vi "Chrg_Dschrg_PTB.vi"(0 "Data Task in":refnum<k21>, 1 "data task error in":errorcluster, 2 "#DAQ outputs (1-13)":i32, 3 "Battery Type":T1(ring), 4 "PS VISA in 2":refnum<visa-resource-name>, 5 "PS error in 2":errorcluster, 6 "CyclePath 2":path=path "C:/Users/ga11/Desktop/VI/results/3PtestCharge.lvm" caption="Filename", 8 "Charge/discharge 2":enum8{"Charge", "Discharge"}(ring), 9 "Charge/Discharge Voltage Setpoint  2":dbl format="%#.6g", 10 "CC or CCCV 2":enum16{"CC", "CCCV"}(ring), 11 "Current Setpoint 2":dbl format="%#.6g", 13 "Current Cutoff 2":dbl) -> (14 "data task out":refnum<k21>, 15 "data task error out":errorcluster, 18 "PS VISA out":refnum<visa-resource-name>, 19 "PS error out 2":errorcluster)   [LabVIEW 2020]
uses:
  IT-M3400/IT-M3400.lvlib
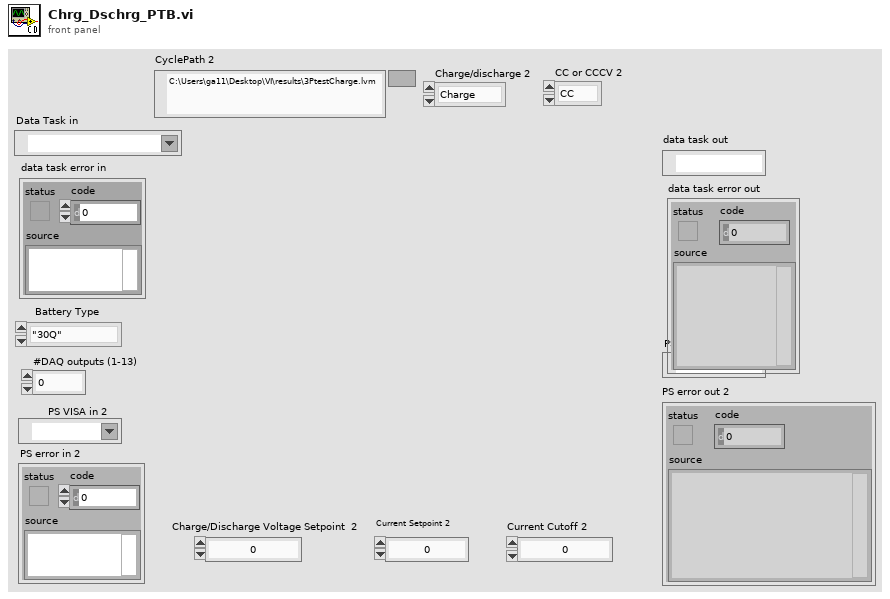
[diagram p1: front panel]
types:
  T1 = enum16{"\"30Q\"", "\"40T\"", "\"2P30Q\"", "\"3P30Q\"", "\"Nissan Leaf\""}
  T2 = cluster{"Baud Rate":u32, "Parity":u16, "Data Bits":u16, "Stop Bits":u16, "Flow Control":u16}
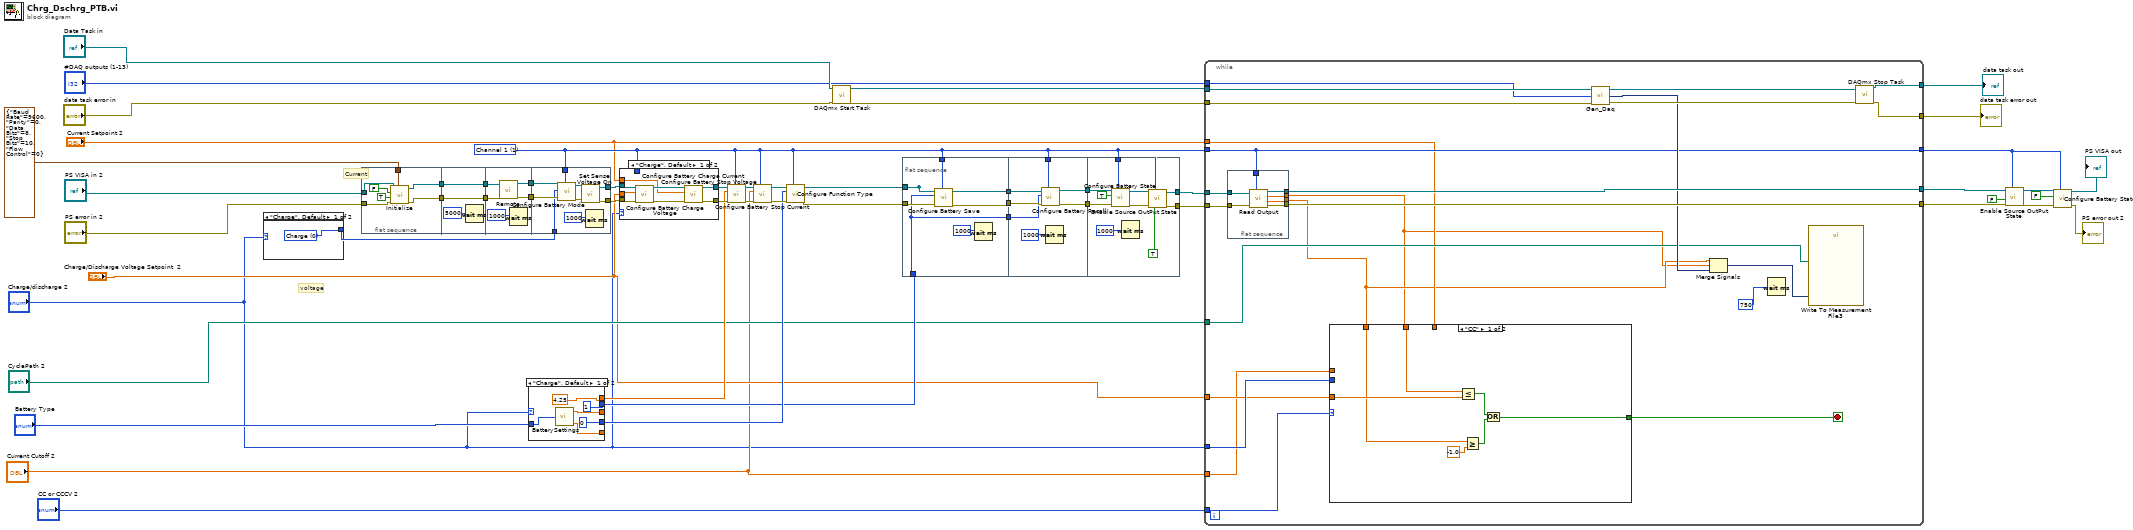
[diagram p0: block diagram]
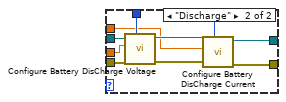
[diagram p2: hidden frame]
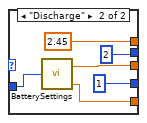
[diagram p3: hidden frame]
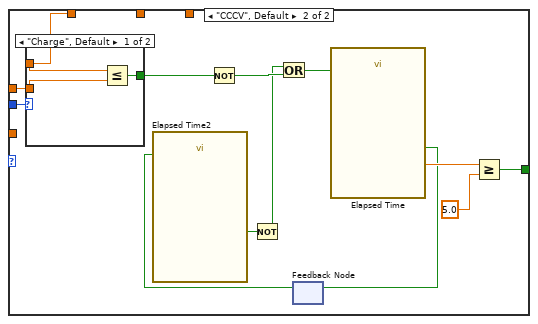
[diagram p4: hidden frame]
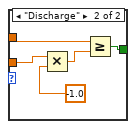
[diagram p5: hidden frame]
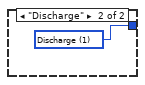
[diagram p6: hidden frame]
diagram:
  w23 = 1 items=["Channel 1"=1, "Channel 2"=2, "Channel 3"=3, "Channel 4"=4, "Channel 5"=5, "Channel 6"=6, "Channel 7"=7, "Channel 8"=8, "Channel 8"=9, "Channel 10"=10, "Channel 11"=11, "Channel 12"=12, "Channel 13"=13, "Channel 14"=14, "Channel 15"=15, "Channel 16"=16] ("Channel")
  # "voltage"
  # "Current"
  n1 = case shown="\"Charge\", Default" "Charge/discharge 2" {
    tunnel: [w55 w56] -> w28
    frame "Charge", Default {
      w55 = u8 0 items=["Charge", "Discharge"] ("Battery Mode")
    }
    frame "Discharge" {
      w56 = u8 1 items=["Charge", "Discharge"] ("Battery Mode")
    }
  }
  n2 = flat-sequence {
    tunnel: [w59] -> w49
    tunnel: [w60] -> w48
    tunnel: T2 {"Baud Rate"=9600, "Parity"=0, "Data Bits"=8, "Stop Bits"=10, "Flow Control"=0} ("Serial Configuration") -> [w63]
    tunnel: "PS error in 2" -> [w62]
    tunnel: "PS VISA in 2" -> [w61]
    tunnel: w49 -> [w66]
    tunnel: [w66] -> w47
    tunnel: w48 -> [w65]
    tunnel: [w65] -> w46
    tunnel: [w71] -> w45
    tunnel: [w70] -> w44
    tunnel: w47 -> [w69]
    tunnel: w46 -> [w68]
    tunnel: w45 -> [w77]
    tunnel: w44 -> [w79]
    tunnel: w23 -> [w80]
    tunnel: w28 -> [w78]
    tunnel: [w72] -> w20
    tunnel: [w73] -> w19
    frame #0 {
      n3 = call "Initialize.vi"("Serial Configuration"=w63, "error in"=w62, "Reset"=TRUE, "ID Query"=FALSE, "VISA resource name"=w61) -> ("error out"=w60:errorcluster, "VISA resource name out"=w59:refnum<visa-resource-name>)  [unwired: 5 in]
    }
    frame #1 {
      n4 = Wait (ms)(milliseconds to wait=5000) -> ()  [unwired: 1 out]
    }
    frame #2 {
      n5 = call "Remote.vi"("error in"=w68, "VISA resource name"=w69) -> ("error out"=w70:errorcluster, "VISA resource name out"=w71:refnum<visa-resource-name>)  [unwired: 8 in]
      n6 = Wait (ms)(milliseconds to wait=1000) -> ()  [unwired: 1 out]
    }
    frame #3 {
      n7 = call "Configure Battery Mode.vi"("Channel"=w80, "error in"=w79, "Battery Mode"=w78, "VISA resource name"=w77) -> ("error out"=w75:errorcluster, "VISA resource name out"=w74:refnum<visa-resource-name>)  [unwired: 6 in]
      n8 = call "Set Sense Voltage On.vi"("error in"=w75, "VISA resource name"=w74) -> ("error out"=w72:errorcluster, "VISA resource name out"=w73:refnum<visa-resource-name>)  [unwired: 8 in]
      n9 = Wait (ms)(milliseconds to wait=1000) -> ()  [unwired: 1 out]
    }
  }
  n10 = case shown="\"Charge\", Default" "Charge/discharge 2" {
    tunnel: [w86 w91] -> _
    tunnel: [u8 0 ("File") u8 1 ("File")] -> w24
    tunnel: [u8 1 ("File") u8 2 ("File")] -> w22
    tunnel: [w83 w89] -> _
    tunnel: [4.25 2.45] -> w21
    tunnel: "Battery Type" -> [w81 w87]
    frame "Charge", Default {
      n11 = call "BatterySettings.vi"("Battery Type"=w81) -> ("RatedCapacity (Ah)"=w83:dbl, "Max Voltage (V)"=w86:dbl)  [unwired: 2 in, 1 out]
    }
    frame "Discharge" {
      n12 = call "BatterySettings.vi"("Battery Type"=w87) -> ("RatedCapacity (Ah)"=w89:dbl, "Min Voltage (V)"=w91:dbl)  [unwired: 2 in, 1 out]
    }
  }
  n13 = case shown="\"Charge\", Default" "Charge/discharge 2" {
    tunnel: w19 -> [w100 w109]
    tunnel: w20 -> [w99 w108]
    tunnel: [w94 w105] -> w35
    tunnel: [w93 w104] -> w34
    tunnel: w23 -> [_ w103]
    tunnel: "Charge/Discharge Voltage Setpoint  2" -> [w96 w102]
    tunnel: "Current Setpoint 2" -> [w95 w101]
    frame "Charge", Default {
      n14 = call "Configure Battery Charge Voltage.vi"("error in"=w99, "Charge Voltage(V)"=w96, "VISA resource name"=w100) -> ("error out"=w97:errorcluster, "VISA resource name out"=w98:refnum<visa-resource-name>)  [unwired: 6 in]
      n15 = call "Configure Battery Charge Current.vi"("error in"=w97, "Charge Current(A)"=w95, "VISA resource name"=w98) -> ("error out"=w93:errorcluster, "VISA resource name out"=w94:refnum<visa-resource-name>)  [unwired: 7 in]
    }
    frame "Discharge" {
      n16 = call "Configure Battery DisCharge Voltage.vi"("Channel"=w103, "error in"=w108, "Discharge Voltage(V)"=w102, "VISA resource name"=w109) -> ("error out"=w106:errorcluster, "VISA resource name out"=w107:refnum<visa-resource-name>)  [unwired: 6 in]
      n17 = call "Configure Battery DisCharge Current.vi"("Channel"=w103, "error in"=w106, "Discharge Current(A)"=w101, "VISA resource name"=w107) -> ("error out"=w104:errorcluster, "VISA resource name out"=w105:refnum<visa-resource-name>)  [unwired: 6 in]
    }
  }
  n18 = call "Configure Battery Stop Voltage.vi"("Channel"=w23, "error in"=w34, "Stop Voltage(V)"=w21, "VISA resource name"=w35) -> ("error out"=w40:errorcluster, "VISA resource name out"=w41:refnum<visa-resource-name>)  [unwired: 6 in]
  n19 = call "Configure Battery Stop Current.vi"("Channel"=w23, "error in"=w40, "Stop Current(A)"="Current Cutoff 2", "VISA resource name"=w41) -> ("error out"=w25:errorcluster, "VISA resource name out"=w26:refnum<visa-resource-name>)  [unwired: 6 in]
  n20 = call "Configure Function Type.vi"("Channel"=w23, "error in"=w25, "Function Type"=w24, "VISA resource name"=w26) -> ("error out"=w1:errorcluster, "VISA resource name out"=w2:refnum<visa-resource-name>)  [unwired: 6 in]
  n21 = call <vilib>:"DAQmx Start Task.vi"("task/channels in"="Data Task in", "error in"="data task error in") -> ("task out"=w15:refnum<k21>, "error out"=w16:errorcluster)  [unwired: 12 in]
  n22 = flat-sequence {
    tunnel: w22 -> [w115]
    tunnel: w23 -> [w111]
    tunnel: [w114] -> w54
    tunnel: [w115] -> w53
    tunnel: [w113] -> w52
    tunnel: w1 -> [w116]
    tunnel: [w110] -> _
    tunnel: w2 -> [w110]
    tunnel: [w119] -> w51
    tunnel: [w120] -> w50
    tunnel: w54 -> [w123]
    tunnel: w53 -> [w122]
    tunnel: w52 -> [w121]
    tunnel: w23 -> [w117]
    tunnel: [w127] -> w33
    tunnel: [w126] -> w32
    tunnel: w23 -> [w125]
    tunnel: w51 -> [w133]
    tunnel: w50 -> [w132]
    frame #0 {
      n23 = call "Configure Battery Save.vi"("Channel"=w111, "error in"=w116, "File"=w115, "VISA resource name"=w110) -> ("error out"=w114:errorcluster, "VISA resource name out"=w113:refnum<visa-resource-name>)  [unwired: 6 in]
      n24 = Wait (ms)(milliseconds to wait=1000) -> ()  [unwired: 1 out]
    }
    frame #1 {
      n25 = call "Configure Battery Recall.vi"("Channel"=w117, "error in"=w123, "File"=w122, "VISA resource name"=w121) -> ("error out"=w120:errorcluster, "VISA resource name out"=w119:refnum<visa-resource-name>)  [unwired: 6 in]
      n26 = Wait (ms)(milliseconds to wait=1000) -> ()  [unwired: 1 out]
    }
    frame #2 {
      n27 = call "Configure Battery State.vi"("Channel"=w125, "error in"=w132, "State"=TRUE, "VISA resource name"=w133) -> ("error out"=w130:errorcluster, "VISA resource name out"=w131:refnum<visa-resource-name>)  [unwired: 6 in]
      n28 = Wait (ms)(milliseconds to wait=1000) -> ()  [unwired: 1 out]
      n29 = call "Enable Source OutPut State.vi"("Channel"=w125, "error in"=w130, "State"=TRUE ("Enable Output|Intput"), "VISA resource name"=w131) -> ("error out"=w126:errorcluster, "VISA resource name out"=w127:refnum<visa-resource-name>)  [unwired: 6 in]
    }
  }
  n30 = while {
    tunnel: [w157] -> w31
    tunnel: [w156] -> w30
    tunnel: w33 -> [w139]
    tunnel: w32 -> [w138]
    tunnel: w23 -> [w140]
    tunnel: [w140] -> w29
    tunnel: "CyclePath 2" -> [w145]
    tunnel: "Charge/discharge 2" -> [w147]
    tunnel: w16 -> [w150]
    tunnel: w15 -> [w149]
    tunnel: "#DAQ outputs (1-13)" -> [w148]
    tunnel: "CC or CCCV 2" -> [w146]
    tunnel: "Charge/Discharge Voltage Setpoint  2" -> [w144]
    tunnel: "Current Cutoff 2" -> [w143]
    tunnel: [w142] -> w9
    tunnel: [w141] -> w8
    tunnel: "Current Setpoint 2" -> [w137]
    stop <- w136 stop-if-true
    n31 = flat-sequence {
      tunnel: [w160] -> w134
      tunnel: [w161] -> w135
      tunnel: [w162] -> w156
      tunnel: [w159] -> w157
      tunnel: w140 -> [w164]
      tunnel: w139 -> [w163]
      tunnel: w138 -> [w158]
      frame #0 {
        n32 = call "Read Output.vi"("Channel"=w164, "error in"=w158, "VISA resource name"=w163) -> ("error out"=w162:errorcluster, "Read Current(A)"=w161:dbl, "Read Voltage(V)"=w160:dbl, "VISA resource name out"=w159:refnum<visa-resource-name>)  [unwired: 5 in]
      }
    }
    n33 = case shown="\"CC\"" w146 {
      tunnel: [w166 w178] -> w136
      tunnel: w143 -> [_ w175]
      tunnel: w134 -> [w171 _]
      tunnel: w144 -> [w170 _]
      tunnel: w147 -> [_ w173]
      tunnel: w135 -> [w169 w172]
      tunnel: w137 -> [_ _]
      frame "CC" {
        n34 = Less Or Equal?(x=w171, y=w170) -> (x <= y?=w167:bool)
        n35 = Greater Or Equal?(x=w169, y=-1.0) -> (x >= y?=w168:bool)
        n36 = Or(x=w167, y=w168) -> (x .or. y?=w166:bool)
      }
      frame "CCCV", Default {
        n37 = case shown="\"Charge\", Default" w173 {
          tunnel: w175 -> [w186 w191]
          tunnel: w172 -> [w187 w189]
          tunnel: [w185 w188] -> w174
          frame "Charge", Default {
            n38 = Less Or Equal?(x=w187, y=w186) -> (x <= y?=w185:bool)
          }
          frame "Discharge" {
            n39 = Multiply(x=w191, y=-1.0) -> (x*y=w190:dbl)
            n40 = Greater Or Equal?(x=w189, y=w190) -> (x >= y?=w188:bool)
          }
        }
        n41 = Not(x=w174) -> (.not. x?=w184:bool)
        n42 = feedback #1() -> (w176:bool)  [unwired: 1 in]
        n43 = call "Elapsed Time2"("Reset"=w176) -> ("Time has Elapsed"=w183:bool)  [unwired: 11 in, 7 out]
        n44 = Not(x=w183) -> (.not. x?=w182:bool)
        n45 = Or(x=w182, y=w184) -> (x .or. y?=w181:bool)
        n46 = call "Elapsed Time"("Reset"=w181) -> ("Elapsed Time (s)"=w180:dbl, "Time has Elapsed"=w177:bool)  [unwired: 11 in, 6 out]
        n47 = feedback-in #1(w177) -> ()
        n48 = Greater Or Equal?(x=w180, y=5.0) -> (x >= y?=w178:bool)
      }
    }
    n49 = call "Gen_Daq.vi"("error in"=w150, "#DAQ outputs (1-13)"=w148, "task/channels in"=w149) -> ("error out"=w152:errorcluster, "DaQ_output"=w151:dynamicdata, "task out"=w153:refnum<k21>)
    n50 = Merge Signals "Merge Signals"(w135, w134, w151) -> (w155:dynamicdata)
    n51 = Wait (ms)(milliseconds to wait=750) -> ()  [unwired: 1 out]
    n52 = call "Write To Measurement File3"("Signals"=w155, "Filename"=w145) -> ()  [unwired: 15 in, 3 out]
    n53 = call <vilib>:"DAQmx Stop Task.vi"("task/channels in"=w153, "error in"=w152) -> ("task out"=w142:refnum<k21>, "error out"=w141:errorcluster)  [unwired: 12 in]
  }
  "data task out" <- w9
  "data task error out" <- w8
  n54 = call "Enable Source OutPut State.vi"("Channel"=w29, "error in"=w30, "State"=FALSE, "VISA resource name"=w31) -> ("error out"=w38:errorcluster, "VISA resource name out"=w39:refnum<visa-resource-name>)  [unwired: 6 in]
  n55 = call "Configure Battery State.vi"("Channel"=w29, "error in"=w38, "State"=FALSE, "VISA resource name"=w39) -> ("error out"=→"PS error out 2":errorcluster, "VISA resource name out"=→"PS VISA out":refnum<visa-resource-name>)  [unwired: 6 in]
